vi "Lossy Enqueue Probe NI.vi"(0 "first":string, 5 "second":string, 11 "error in":errorcluster) -> (4 "overflow element":string, 6 "overflow?":bool, 8 "remaining elements":string[](array[string]), 15 "error out":errorcluster)   [LabVIEW 2026]
doc: "Probe: a size-1 queue takes first, then second through Lossy Enqueue Element; the second overflows first out."
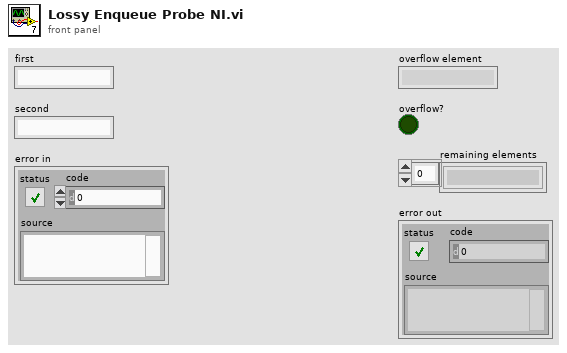
[diagram p1: front panel]
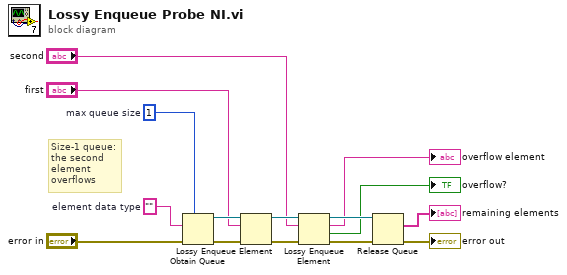
[diagram p0: block diagram]
diagram:
  w14 = 1  # max queue size
  w15 = ""  # element data type
  # "Size-1 queue: the second element overflows"
  n1 = Obtain Queue(max queue size (-1, unlimited)=w14, element data type=w15, error in (no error)="error in") -> (queue out=w12:refnum<queue>, error out=w10:errorcluster)  [unwired: 2 in, 1 out]
  n2 = Lossy Enqueue Element(queue=w12, element="first", error in (no error)=w10) -> (queue out=w9:refnum<queue>, error out=w7:errorcluster)  [unwired: 2 out]
  n3 = Lossy Enqueue Element(queue=w9, element="second", error in (no error)=w7) -> (queue out=w6:refnum<queue>, overflow element=→"overflow element":string, overflow?=→"overflow?":bool, error out=w5:errorcluster)
  n4 = Release Queue(queue=w6, error in (no error)=w5) -> (remaining elements=→"remaining elements":string[], error out=→"error out":errorcluster)  [unwired: 1 in, 1 out]
